vi "FX232_485_BWWW.vi"(4 "值":string, 5 "延时":u8 max=150 step=10, 6 "数量":u8=1, 7 "PLC站号":u8=1, 8 "error in (no error)":errorcluster caption="错误输入（无错误）", 9 "地址":string, 10 "命令":string(combo), 11 "Port":refnum<visa-resource-name>) -> (0 "error out":errorcluster caption="错误输出", 1 "成功":bool, 2 "Buff":string, 3 "PortOut":refnum<visa-resource-name>)   [LabVIEW 2025]
uses:
  <vilib>/Utility/error.llb/Trim Whitespace One-Sided.vi
panel:
  out "连接的字符串":string
  # "Y,D,M"
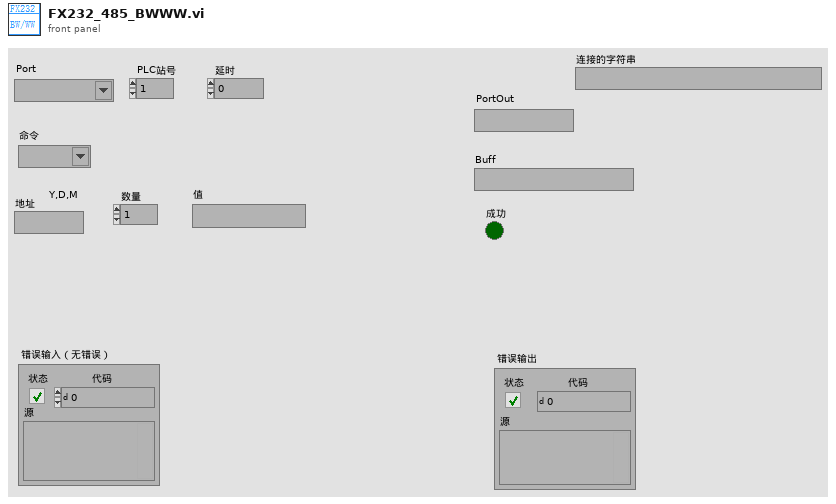
[diagram p1: front panel]
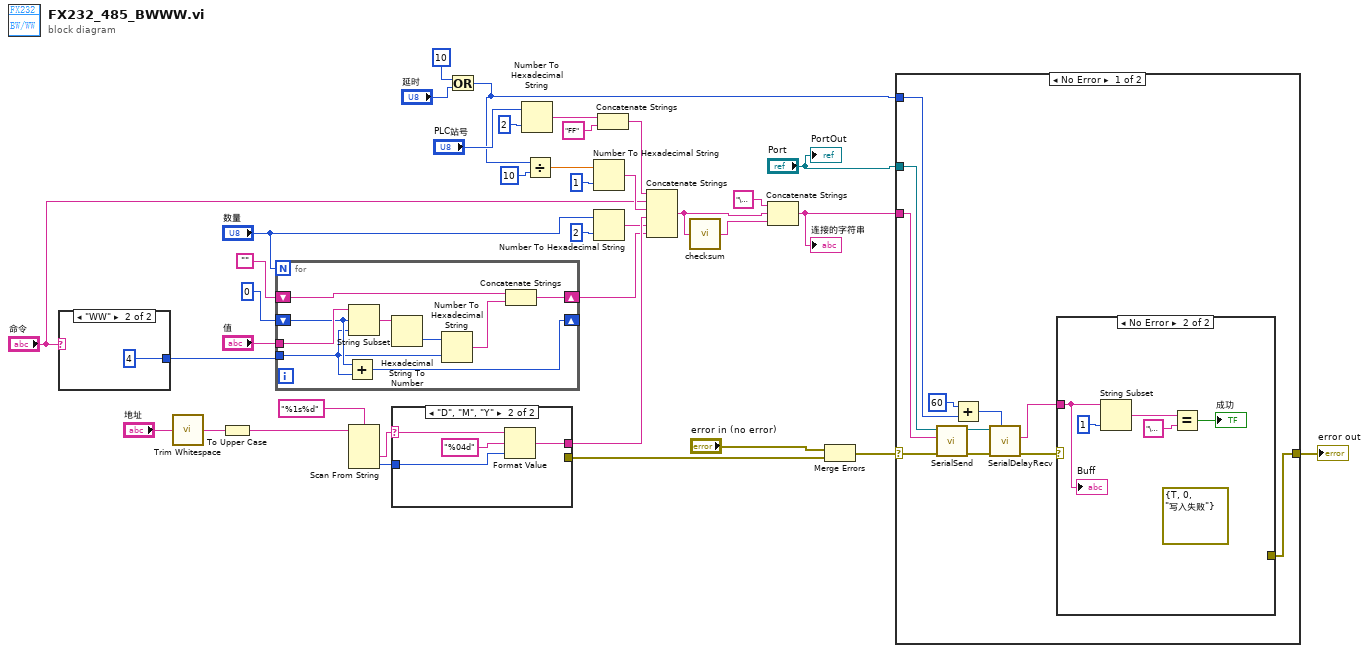
[diagram p0: block diagram]
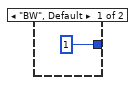
[diagram p2: hidden frame]
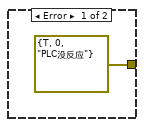
[diagram p3: hidden frame]
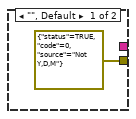
[diagram p5: hidden frame]
diagram:
  n1 = case shown="\"WW\"" "命令" {
    tunnel: [1 4] -> w5
    frame "BW", Default {
    }
    frame "WW" {
    }
  }
  n2 = call <vilib>:"Trim Whitespace.vi"("string"="地址") -> ("trimmed string"=w33:string)  [unwired: 1 in]
  n3 = To Upper Case(1:w33) -> (0:w35:string)
  n4 = for {
    N: "数量" -> [_]
    tunnel: "值" -> [w48]
    tunnel: w5 -> [w44]
    shift-right: [w43] -> _
    shift-left: 0 -> [w45]
    shift-right: [w40] -> w12
    shift-left: "" -> [w42]
    n5 = Add(x=w45, y=w44) -> (x+y=w43:i32)
    n6 = String Subset(string=w48, offset (0)=w45, length (rest)=w44) -> (substring=w47:string)
    n7 = Hexadecimal String To Number(string=w47) -> (number=w46:u32)  [unwired: 2 in, 1 out]
    n8 = Number To Hexadecimal String(1:w44, 2:w46) -> (0:w41:string)
    n9 = Concatenate Strings(w42, w41) -> (w40:string)
  }
  n10 = Scan From String(format string="%1s%d" ("格式字符串"), input string=w35) -> (output 1=w36:string, output 2=w32:i32)  [unwired: 4 in, 3 out]
  n11 = case shown="\"D\", \"M\", \"Y\"" w36 {
    selector: w36 -> [_ w53]
    tunnel: w32 -> [_ w51]
    tunnel: [errorcluster {"status"=TRUE, "code"=0, "source"="Not Y,D,M"} ("error in (no error)") _] -> w7
    tunnel: [_ w50] -> w25
    frame "", Default {
    }
    frame "D", "M", "Y" {
      n12 = Format Value(string ("")=w53, format string="%04d" ("格式字符串"), value (0)=w51) -> (output string=w50:string)
    }
  }
  n13 = Or(x=10, y="延时") -> (x .or. y?=w2:i32)
  n14 = Number To Hexadecimal String(1:i16 2 ("宽度(-)"), 2:"PLC站号") -> (0:w23:string)
  n15 = Divide(x=w2, y=10) -> (x/y=w27:dbl)
  n16 = Number To Hexadecimal String(1:i16 1 ("宽度(-)"), 2:w27) -> (0:w22:string)
  n17 = Number To Hexadecimal String(1:i16 2 ("宽度(-)"), 2:"数量") -> (0:w11:string)
  n18 = Concatenate Strings(w23, "FF" ("字符串")) -> (w20:string)
  n19 = Concatenate Strings(w20, "命令", w22, w25, w11, w12) -> (w17:string)
  n20 = call "checksum.vi"("buff"=w17) -> ("checksum"=w16:string)  [unwired: 4 in]
  n21 = Concatenate Strings("\u0005" ("字符串"), w17, w16) -> (w26:string)
  "连接的字符串" <- w26
  n22 = Merge Errors("error in (no error)", w7) -> (w6:errorcluster)
  n23 = case shown="No Error" w6 {
    selector: w6 -> [w62 w71]
    tunnel: w26 -> [w64 _]
    tunnel: "Port" -> [w63 _]
    tunnel: [w61 w71] -> w31
    tunnel: w2 -> [w60 _]
    frame No Error {
      n24 = call "SerialSend.vi"("error in (no error)"=w62, "SendData"=w64, "PORT"=w63) -> ("error out"=w56:errorcluster, "PORT out"=w58:refnum<visa-resource-name>)  [unwired: 6 in, 1 out]
      n25 = Add(x=u32 60 ("等待时间（毫秒）"), y=w60) -> (x+y=w57:u32)
      n26 = call "SerialDelayRecv.vi"("Timeout"=w57, "error in (no error)"=w56, "Port"=w58) -> ("error out"=w54:errorcluster, "Buff"=w55:string)  [unwired: 6 in, 1 out]
      n27 = case shown="No Error" w54 {
        tunnel: [errorcluster {"status"=TRUE, "code"=0, "source"="PLC没反应"} ("错误常量") _] -> w61
        tunnel: w55 -> [_ w67]
        frame Error {
        }
        frame No Error {
          (unwired) errorcluster {"status"=TRUE, "code"=0, "source"="写入失败"} ("错误常量")
          n28 = String Subset(string=w67, length (rest)=1 ("长度（剩余）")) -> (substring=w69:string)  [unwired: 1 in]
          n29 = Equal?(x=w69, y="\u0006") -> (x = y?=→"成功":bool)
          "Buff" <- w67
        }
      }
    }
    frame Error {
    }
  }
  "error out" <- w31
  "PortOut" <- "Port"
